vi "GMAP_API_Get_route (SubVI).vi"(8 "error in (no error)":errorcluster, 9 "Route speed, mph":dbl, 10 "Route altitude, feet":dbl, 11 "Browser control ref in":refnum<vi>) -> (0 "error out":errorcluster, 1 "Coordinates string (out)":string, 2 "Coordinates":string, 3 "Browser control ref out":refnum<vi>)   [LabVIEW 2025]
doc: "This VI gets route waypoints coordinates\nfrom Google map using Javascript request"
uses:
  <vilib>/sklein/WebView2 XControl/WebView2 XControl/WebView2 Control.xctl
panel:
  # "This VI gets route waypoints coordinates\nfrom Google map using Javascript request"
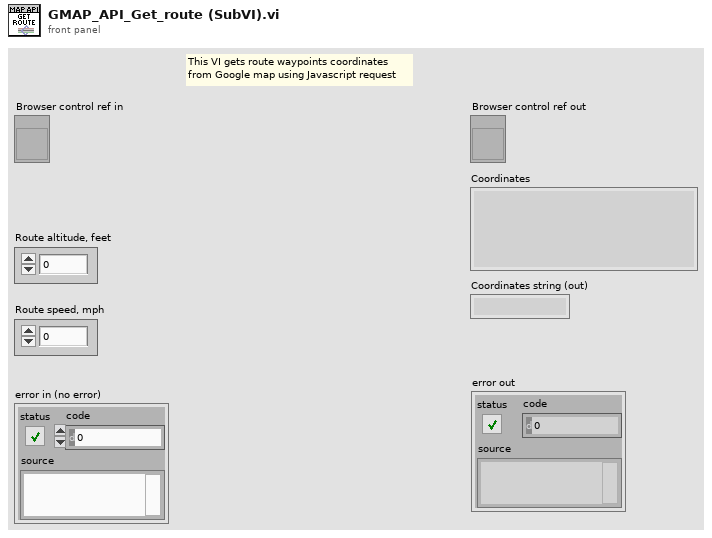
[diagram p1: front panel]
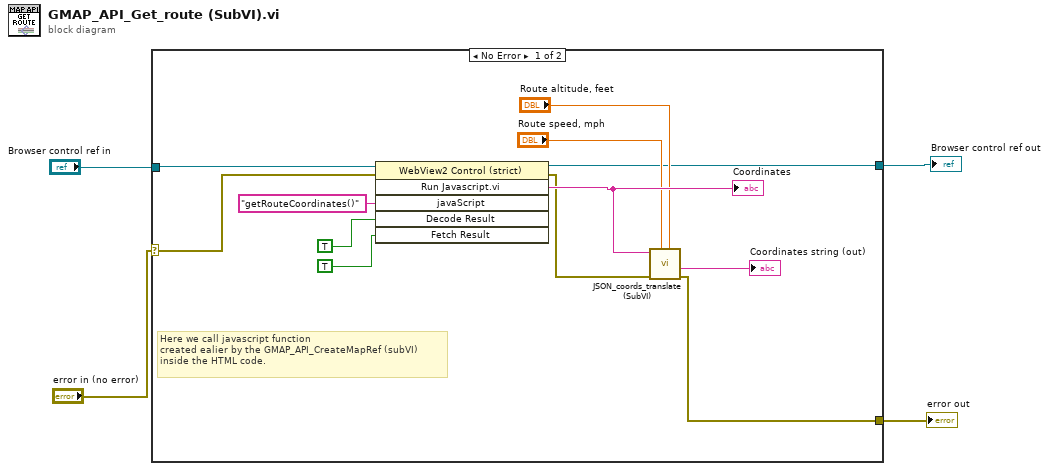
[diagram p0: block diagram]
diagram:
  n1 = case shown="No Error" "error in (no error)" {
    selector: "error in (no error)" -> [w8 w18]
    tunnel: [w5 w18] -> w4
    tunnel: "Browser control ref in" -> [w9 w17]
    tunnel: [w7 w17] -> w1
    frame No Error {
      # "Here we call javascript function\ncreated ealier by the GMAP_API_CreateMapRef (subVI)\ninside the HTML code."
      n2 = invoke class="WebView2 Control (strict)" method="Run Javascript.vi"(reference=w9, error in=w8, "javaScript"="getRouteCoordinates()", "Decode Result"=TRUE, "Fetch Result"=TRUE) -> (reference out=w7:refnum<vi>, error out=w6:errorcluster, "Run Javascript.vi"=w16:string)  [unwired: 1 in, 3 out]
      "Coordinates" <- w16
      n3 = call "JSON_coords_translate (SubVI).vi"("Altitude, m"="Route altitude, feet", "Speed, mph"="Route speed, mph", "error in"=w6, "Coordinates string (in)"=w16) -> ("error out"=w5:errorcluster, "Coordinates string (out)"=→"Coordinates string (out)":string)  [unwired: 5 in, 1 out]
    }
    frame Error {
    }
  }
  "error out" <- w4
  "Browser control ref out" <- w1
